vi "UE_Run_Id_Matches.vi"(1 "active_run_id":i32, 2 "incoming_run_id":i32) -> (0 "same_run":bool)   [LabVIEW 2026]
doc: "INTENT: Reject a stale command or result whose integer demonstration run identifier differs. INPUTS: incoming_run_id (int32), active_run_id (int32). OUTPUTS: same_run (bool). DESIGN CONSTRAINT: Production run IDs should use stronger unique identities; this is only a comparison helper. REQUIREMENTS: SRS-F-024. No physical hardware side effects. Acceptance requires native LabVIEW compilation and behavioral testing."
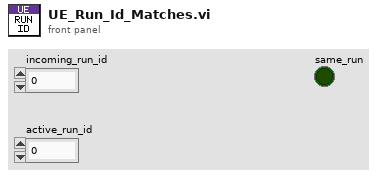
[diagram p1: front panel]
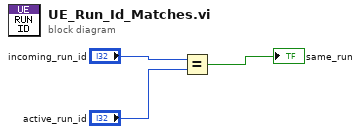
[diagram p0: block diagram]
diagram:
  n1 = Equal?(x="incoming_run_id", y="active_run_id") -> (x = y?=→"same_run":bool)
